vi "zadanie_4_lab0.vi"() -> ()   [LabVIEW 2020]
uses:
  <vilib>/numeric/Random Number (Range) U64.vi
  <vilib>/numeric/sub_Random U32.vi
panel:
  in  "error in":errorcluster
  out "error out":errorcluster
  out "Tablicza porównawcza":bool[](array[boolean])
  in  "Zadana liczba wykonañ programu":i32
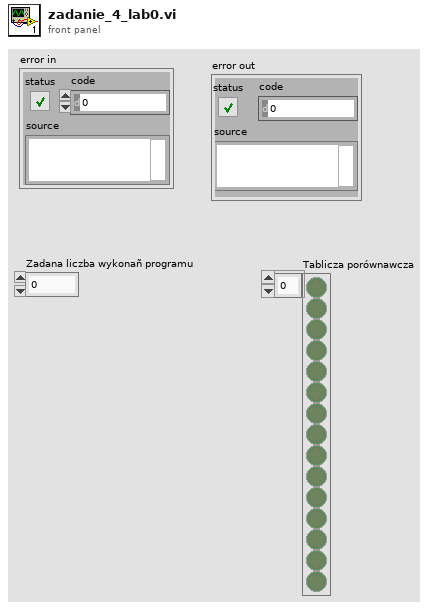
[diagram p1: front panel]
types:
  T1 = enum16{"open", "replace", "create", "open or create", "replace or create", "replace or create with confirmation"}
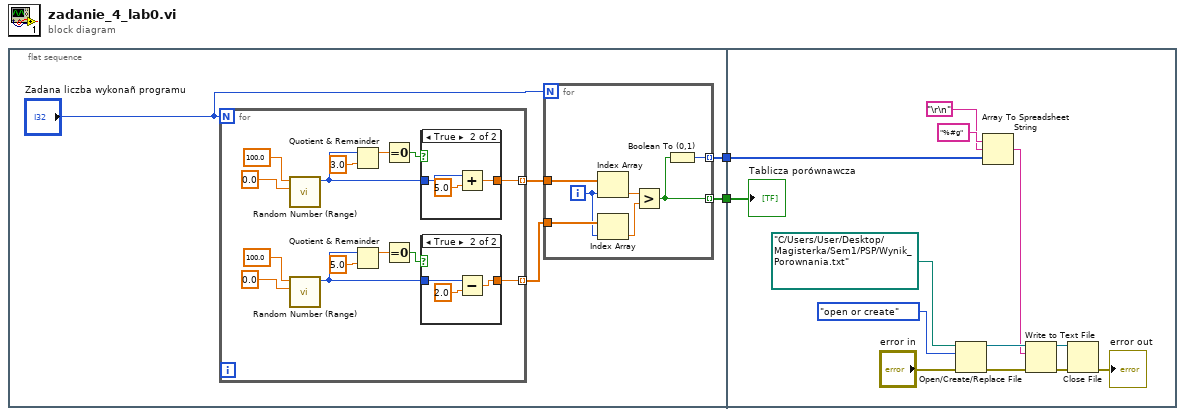
[diagram p0: block diagram]
diagram:
  n1 = flat-sequence {
    tunnel: [w4] -> w2
    tunnel: [w3] -> w1
    tunnel: w2 -> [w41]
    tunnel: w1 -> [w40]
    frame #0 {
      n2 = for {
        N: "Zadana liczba wykonañ programu" -> [_]
        tunnel: [w17] -> w7 mode=indexing
        tunnel: [w15] -> w6 mode=indexing
        n3 = call-poly <vilib>:"Random Number (Range).vi"("lower bound (0)"=0.0, "upper bound (100)"=100.0) -> ("number"=w18:u64)  [unwired: 9 in]
        n4 = call-poly <vilib>:"Random Number (Range).vi"("lower bound (0)"=0.0, "upper bound (100)"=100.0) -> ("number"=w16:u64)  [unwired: 9 in]
        n5 = Quotient & Remainder(x=w18, y=3.0) -> (x-y*floor(x/y)=w22:dbl)  [unwired: 1 out]
        n6 = Quotient & Remainder(x=w16, y=5.0) -> (x-y*floor(x/y)=w20:dbl)  [unwired: 1 out]
        n7 = Equal To 0?(x=w22) -> (x = 0?=w21:bool)
        n8 = Equal To 0?(x=w20) -> (x = 0?=w19:bool)
        n9 = case shown="True" w21 {
          tunnel: w18 -> [w29 w32]
          tunnel: [w29 w30] -> w17
          frame False {
          }
          frame True {
            n10 = Add(x=w32, y=5.0) -> (x+y=w30:dbl)
          }
        }
        n11 = case shown="True" w19 {
          tunnel: w16 -> [w33 w36]
          tunnel: [w33 w34] -> w15
          frame False {
          }
          frame True {
            n12 = Subtract(x=w36, y=2.0) -> (x-y=w34:dbl)
          }
        }
      }
      n13 = for {
        N: "Zadana liczba wykonañ programu" -> [_]
        tunnel: w7 -> [w14]
        tunnel: w6 -> [w12]
        tunnel: [w9] -> w4 mode=indexing
        tunnel: [w8] -> w3 mode=indexing
        i -> [w10]
        n14 = Index Array(array=w14, index=w10) -> (element=w13:dbl)
        n15 = Index Array(array=w12, index=w10) -> (element=w11:dbl)
        n16 = Greater?(x=w13, y=w11) -> (0:w9:bool)
        n17 = Boolean To (0,1)(Boolean=w9) -> (0, 1=w8:i16)
      }
    }
    frame #1 {
      n18 = Open/Create/Replace File(file path (use dialog)=path "C:/Users/User/Desktop/Magisterka/Sem1/PSP/Wynik_Porownania.txt", error in="error in", operation (0:open)=T1."open or create") -> (refnum out=w45:refnum<file>, error out=w43:errorcluster)  [unwired: 3 in, 1 out]
      n19 = Array To Spreadsheet String(delimiter (Tab)="\r\n", array=w40, 3:"%#g" ("format string")) -> (spreadsheet string=w39:string)
      n20 = Write to Text File(file (use dialog)=w45, text=w39, error in=w43) -> (refnum out=w44:refnum<file>, error out=w42:errorcluster)  [unwired: 1 in, 1 out]
      n21 = Close File(refnum=w44, error in=w42) -> (error out=→"error out":errorcluster)  [unwired: 1 out]
      "Tablicza porównawcza" <- w41
    }
  }
